vi "PathCal.vi"(9 "pose_y":dbl=7988.0, 10 "pose_x":dbl=8250.0, 11 "语音命令数组":string[][](array[string])) -> (2 "Local_Goal":T1, 3 "Goal_Path":dbl[][](array[numeric]))   [LabVIEW 2014]
uses:
  ctl/Point.ctl
panel:
  out "行数":i32
  out "Path 2":string[](array[string])
  out "Area 3":string[](array[string])
  out "Dis 2":dbl
  out "Path坐标数组":dbl[][](array[numeric])
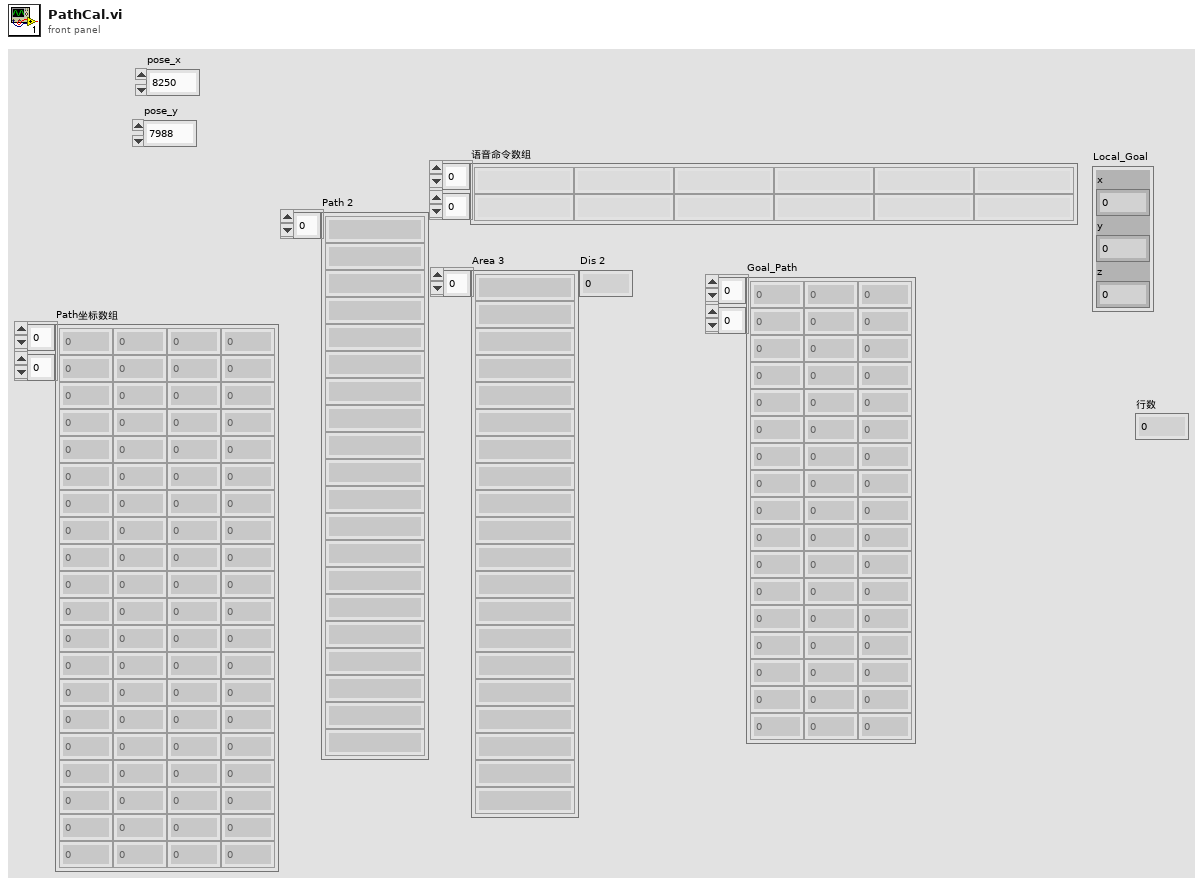
[diagram p1: front panel]
types:
  T1 = typedef "Point.ctl" = cluster{"x":dbl, "y":dbl, "z":dbl}
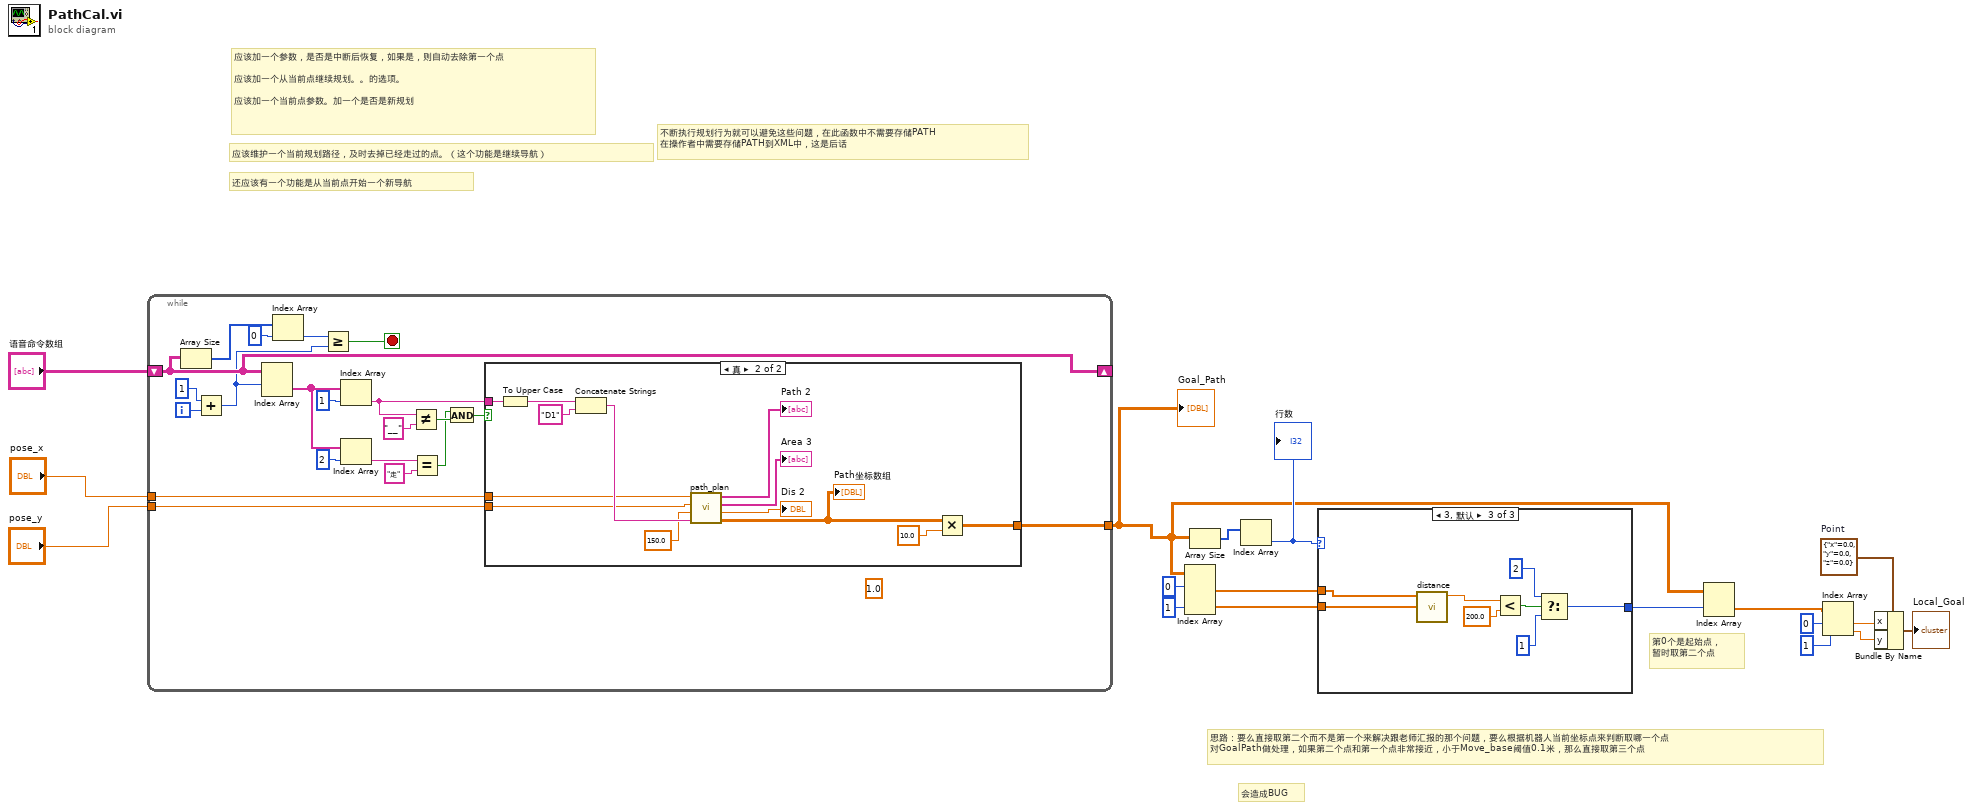
[diagram p0: block diagram]
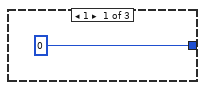
[diagram p2: hidden frame]
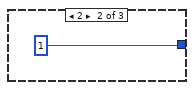
[diagram p3: hidden frame]
diagram:
  w10 = T1 {"x"=0.0, "y"=0.0, "z"=0.0}  # Point
  # "会造成BUG"
  # "第0个是起始点，\n暂时取第二个点"
  # "思路：要么直接取第二个而不是第一个来解决跟老师汇报的那个问题，要么根据机器人当前坐标点来判断取哪一个点\n对GoalPath做处理，如果第二个点和第一个点非常接近，小于Move_base阈值0.1米，那么直接取第三个点"
  # "不断执行规划行为就可以避免这些问题，在此函数中不需要存储PATH\n在操作者中需要存储PATH到XML中，这是后话"
  # "还应该有一个功能是从当前点开始一个新导航"
  # "应该维护一个当前规划路径，及时去掉已经走过的点。（这个功能是继续导航）"
  # "应该加一个参数，是否是中断后恢复，如果是，则自动去除第一个点\n\n应该加一个从当前点继续规划。。的选项。\n\n应该加一个当前点参数。加一个是否是新规划"
  n1 = while {
    shift-right: [w35] -> _
    shift-left: "语音命令数组" -> [w35]
    tunnel: [w21] -> w5
    tunnel: "pose_x" -> [w20]
    tunnel: "pose_y" -> [w19]
    i -> [w37]
    stop <- w34 stop-if-true
    (unwired) 1.0
    n2 = Array Size(array=w35) -> (size(s)=w39:i32[])
    n3 = Add(x=1, y=w37) -> (x+y=w32:i32)
    n4 = Index Array(array=w35, index (row)=w32) -> (element=w27:string[])  [unwired: 1 in]
    n5 = Index Array(array=w39, index=0 ("索引")) -> (element=w33:i32)
    n6 = Greater Or Equal?(x=w33, y=w32) -> (x >= y?=w34:bool)
    n7 = Index Array(array=w27, index=1 ("索引")) -> (element=w22:string)
    n8 = Index Array(array=w27, index=2 ("索引")) -> (element=w30:string)
    n9 = Not Equal?(x=w22, y="__") -> (x != y?=w25:bool)
    n10 = Equal?(x=w30, y="走") -> (x = y?=w24:bool)
    n11 = And(x=w24, y=w25) -> (x .and. y?=w23:bool)
    n12 = case shown="真" w23 {
      tunnel: w22 -> [_ w52]
      tunnel: [_ w43] -> w21
      tunnel: w20 -> [_ w42]
      tunnel: w19 -> [_ w41]
      frame False {
      }
      frame True {
        n13 = To Upper Case(1:w52) -> (0:w51:string)
        n14 = Concatenate Strings(w51, "D1" ("字符串")) -> (w49:string)
        n15 = call "path_plan.vi"("Node2"=w49, "z"=150.0, "y"=w41, "x"=w42) -> ("Path坐标数组"=w44:dbl[][], "Dis 2"=→"Dis 2":dbl, "Area 3"=→"Area 3":string[], "Path 2"=→"Path 2":string[])
        "Path坐标数组" <- w44
        n16 = Multiply(x=w44, y=10.0) -> (x*y=w43:dbl[][])
      }
    }
  }
  "Goal_Path" <- w5
  n17 = Index Array(array=w5, index (row) #1=0 ("索引 (行)"), index (row) #2=1 ("索引 (行)")) -> (element #1=w2:dbl[], element #2=w1:dbl[])  [unwired: 2 in]
  n18 = Array Size(array=w5) -> (size(s)=w8:i32[])
  n19 = Index Array(array=w8) -> (element=w7:i32)  [unwired: 1 in]
  "行数" <- w7
  n20 = case shown="3, 默认" w7 {
    tunnel: [0 1 w57] -> w6
    tunnel: w2 -> [_ _ w62]
    tunnel: w1 -> [_ _ w61]
    frame 1 {
    }
    frame 2 {
    }
    frame 3, Default {
      n21 = call "distance.vi"("子数组 2"=w61, "子数组"=w62) -> ("distance"=w60:dbl)  [unwired: 8 in, 1 out]
      n22 = Less?(x=w60, y=200.0) -> (x < y?=w58:bool)
      n23 = Select(t=2, s=w58, f=1) -> (s? t:f=w57:i32)
    }
  }
  n24 = Index Array(array=w5, index (row)=w6) -> (element=w15:dbl[])  [unwired: 1 in]
  n25 = Index Array(array=w15, index #1=0 ("索引"), index #2=1 ("索引")) -> (element #1=w12:dbl, element #2=w11:dbl)
  n26 = Bundle By Name(cluster=w10, "x"=w12, "y"=w11) -> (→"Local_Goal":T1)
